vi "Neopixel_All.vi"(8 "error in (no error)":errorcluster, 10 "Color Box":u32(colorbox), 11 "VISA resource name":refnum<visa-resource-name>) -> (0 "error out":errorcluster, 2 "respuesta":string, 3 "VISA resource name out":refnum<visa-resource-name>)   [LabVIEW 2026]
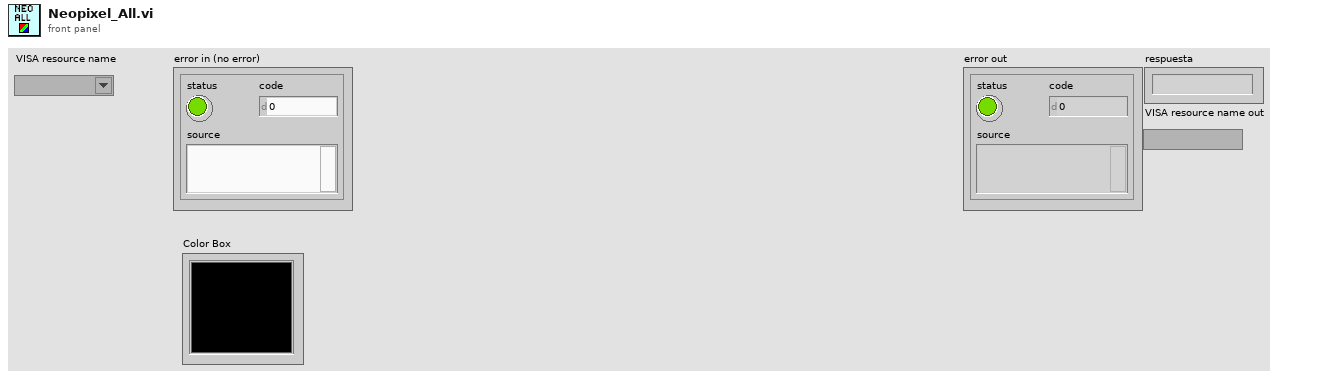
[diagram p1: front panel]
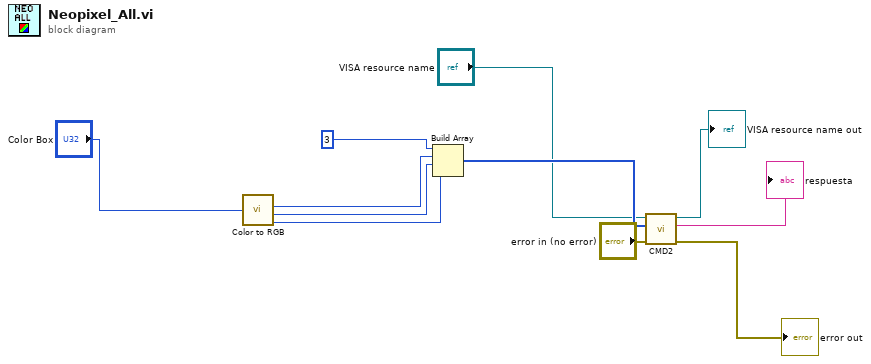
[diagram p0: block diagram]
diagram:
  n1 = call <vilib>:"Color to RGB.vi"("Color"="Color Box") -> ("R"=w9:u8, "G"=w8:u8, "B"=w7:u8)  [unwired: 1 out]
  n2 = Build Array(u8 3, w9, w8, w7) -> (w6:u8[])
  n3 = call "CMD2.vi"("error in (no error)"="error in (no error)", "Comando"=w6, "VISA resource name"="VISA resource name") -> ("error out"=→"error out":errorcluster, "respuesta"=→"respuesta":string, "VISA resource name out"=→"VISA resource name out":refnum<visa-resource-name>)  [unwired: 6 in]
